vi "query NR HO UL_DL Center Channel Numebr.vi"(8 "error in (no error)":errorcluster caption="에러 입력(에러 없음)", 9 "Direction":T2, 10 "Selected CC Argements":T1, 11 "Anritsu Call Box_Implement 입력":refnum<class "Anritsu Call Box_Implement.lvclass">) -> (0 "error out":errorcluster caption="에러 출력", 2 "Center Channel Number":u32, 3 "Anritsu Call Box_Implement 출력":refnum<class "Anritsu Call Box_Implement.lvclass">)   [LabVIEW 2023, in "ANRITSU Call Box.lvlib" / "Anritsu Call Box_Implement.lvclass"]
uses:
  Anritsu Call Box_Implement.lvclass
  Anritsu Call Box_Implement.lvclass/Anritsu Call Box_Implement.ctl
  NR/NR.lvclass
  Type Definition/Uplink Downlink Enum.ctl
  ANRITSU Call Box.lvlib
  Type Definition/NR Selected CC Type Arguments.ctl
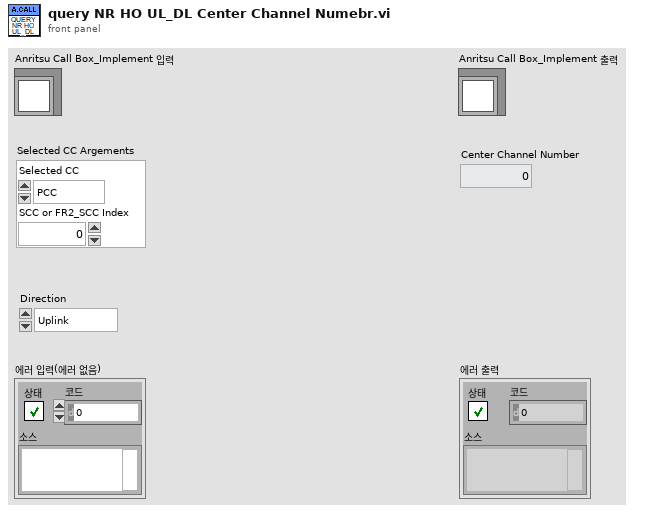
[diagram p1: front panel]
types:
  T1 = typedef "ANRITSU Call Box.lvlib/NR Selected CC Type Arguments.ctl" = cluster{"Selected CC":enum16{"PCC", "SCC", "FR2_PCC", "FR2_SCC"}, "SCC or FR2_SCC Index":u32}
  T2 = typedef "ANRITSU Call Box.lvlib/Uplink Downlink Enum.ctl" = enum16{"Uplink", "Downlink"}
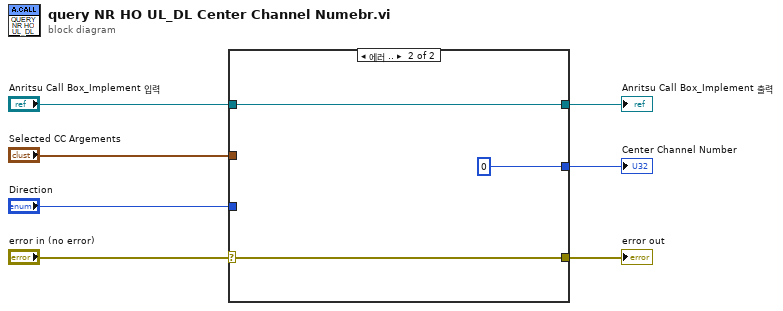
[diagram p0: block diagram]
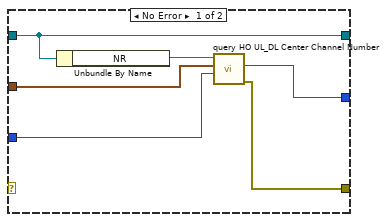
[diagram p2: hidden frame]
diagram:
  n1 = case shown="에러 .." "error in (no error)" {
    selector: "error in (no error)" -> [_ w15]
    tunnel: "Anritsu Call Box_Implement 입력" -> [w13 w16]
    tunnel: [w13 w16] -> w6
    tunnel: [w9 w15] -> w5
    tunnel: "Selected CC Argements" -> [w11 _]
    tunnel: "Direction" -> [w10 _]
    tunnel: [w8 u32 0 ("Center Channel Number")] -> w1
    frame No Error {
      n2 = Unbundle By Name(w13) -> ("NR"=w12:refnum<class "NR.lvclass">)
      n3 = call "query HO UL_DL Center Channel Number.vi"("Direction"=w10, "Selected CC Argements"=w11, "NR 입력"=w12) -> ("error out"=w9:errorcluster, "Center Channel Number"=w8:u32)  [unwired: 6 in, 1 out]
    }
    frame Error {
    }
  }
  "error out" <- w5
  "Anritsu Call Box_Implement 출력" <- w6
  "Center Channel Number" <- w1
